vi "Generate String.vi"(9 "line limit":i32, 10 "log limit":i32, 11 "log buffer":string[](array[string])) -> (2 "indicator string":string, 3 "trimmed log buffer":string[](array[string]))   [LabVIEW 2018, in "GLog.lvlib" / "UI Updater.lvlib"]
uses:
  UI Updater.lvlib
  dependencies/Utilities/Utilities.lvlib
panel:
  # "Connector Pane"
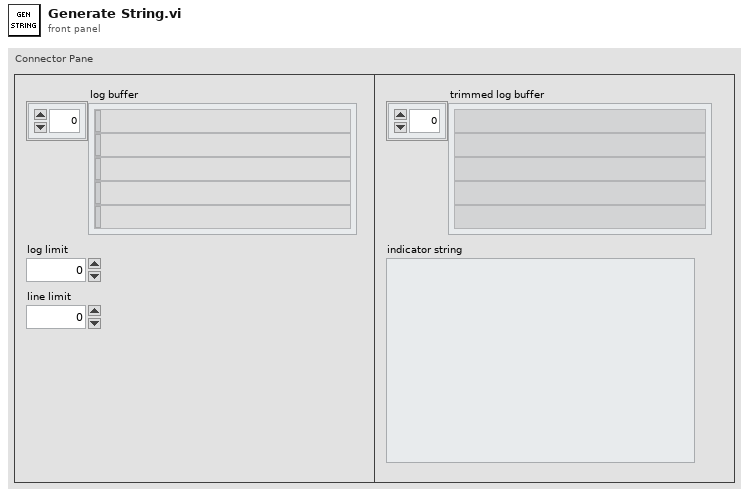
[diagram p1: front panel]
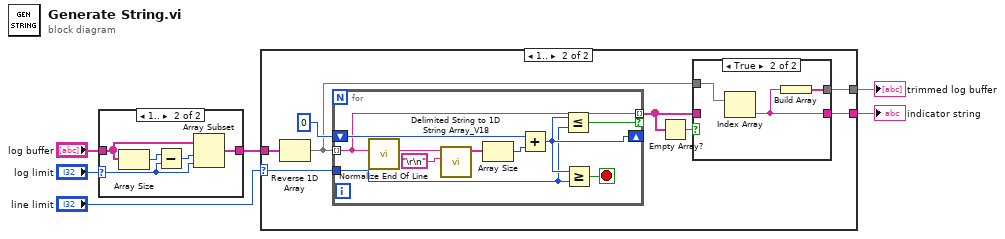
[diagram p0: block diagram]
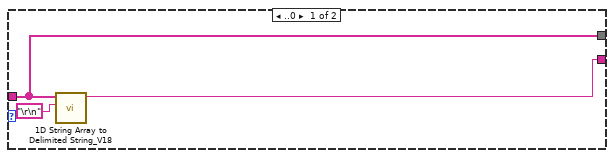
[diagram p2: hidden frame]
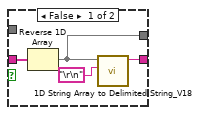
[diagram p3: hidden frame]
diagram:
  n1 = case shown="1.." "log limit" {
    selector: "log limit" -> [_ w9]
    tunnel: "log buffer" -> [w7 w10]
    tunnel: [w7 w8] -> w4
    frame ..0 {
    }
    frame 1.. {
      n2 = Array Size(array=w10) -> (size(s)=w12:i32)
      n3 = Subtract(x=w12, y=w9) -> (x-y=w11:i32)
      n4 = Array Subset(array=w10, index=w11, length=w9) -> (w8:string[])
    }
  }
  n5 = case shown="1.." "line limit" {
    selector: "line limit" -> [_ w21]
    tunnel: w4 -> [w13 w23]
    tunnel: [w14 w17] -> w2
    tunnel: [w13 w16] -> w1
    frame ..0 {
      n6 = call "1D String Array to Delimited String_V18.vi"("delimiter"="\r\n", "string array"=w13) -> ("delimited string"=w14:string)  [unwired: 9 in]
    }
    frame 1.. {
      n7 = Reverse 1D Array(array=w23) -> (reversed array=w19:string[])
      n8 = for {
        tunnel: w19 -> [w29] mode=indexing
        shift-right: [w26] -> _
        shift-left: 0 ("size(s)") -> [w30]
        tunnel: w21 -> [w25]
        tunnel: [w29] -> w18 mode=indexing if=w28
        stop <- w27 stop-if-true
        n9 = call <vilib>:"Normalize End Of Line.vi"("string in"=w29) -> ("string out"=w24:string)  [unwired: 7 in]
        n10 = call "Delimited String to 1D String Array_V18.vi"("delimiter"="\r\n", "delimited string"=w24) -> ("string array"=w32:string[])  [unwired: 9 in]
        n11 = Array Size(array=w32) -> (size(s)=w31:i32)
        n12 = Add(x=w30, y=w31) -> (x+y=w26:i32)
        n13 = Less Or Equal?(x=w26, y=w25) -> (x <= y?=w28:bool)
        n14 = Greater Or Equal?(x=w26, y=w25) -> (x >= y?=w27:bool)
      }
      n15 = Empty Array?(array=w18) -> (empty?=w20:bool)
      n16 = case shown="True" w20 {
        tunnel: w19 -> [_ w40]
        tunnel: w18 -> [w37 _]
        tunnel: [w35 w39] -> w17
        tunnel: [w34 w38] -> w16
        frame False {
          n17 = Reverse 1D Array(array=w37) -> (reversed array=w34:string[])
          n18 = call "1D String Array to Delimited String_V18.vi"("delimiter"="\r\n", "string array"=w34) -> ("delimited string"=w35:string)  [unwired: 9 in]
        }
        frame True {
          n19 = Index Array(array=w40) -> (element=w39:string)  [unwired: 1 in]
          n20 = Build Array(w39) -> (w38:string[])
        }
      }
    }
  }
  "indicator string" <- w2
  "trimmed log buffer" <- w1
